vi "Define Columns.vi"(10 "enum array":refnum<vi>[](array[refnum])) -> (2 "Column Definitions":T1[](array[typedef]) {"MinWidth" min=2 step=1; "AutoSizeMode" items=["None"=1, "ColumnHeader"=2, "AllCellsExceptHeader"=4, "AllCells"=6, "DisplayedCellsExceptHeader"=8, "DisplayedCells"=10, "Fill"=16]; "FillWeight" min=1 max=100})   [LabVIEW 2015, in "Modbus Module editor node.lvclass"]
uses:
  Modbus Module editor node.lvclass
  <vilib>/NI/DCAF/Tag Editor Core/Table API/Column/Column Descriptor.ctl
  <vilib>/NI/DCAF/Tag Editor Core/Table API/Column/Column.lvclass
  <vilib>/NI/DCAF/Tag Editor Core/Table API/Column/Column Type.ctl
  <vilib>/NI/Tag Bus/tag/Data Type.ctl
  <vilib>/NI/DCAF/Tag Editor Core/Table API/Table Manager/Call Back Ref Type Def.ctl
  <vilib>/NI/DCAF/Tag Editor Core/Configuration Editor/Classes/Engine Parent/Engine Parent Editor Node.lvclass
  <vilib>/NI/DCAF/Tag Editor Core/Configuration Editor/Classes/Module editor node/module editor node.lvclass
  Callback Change Direction.vi
  CallBack Change Data Type.vi
  Callback Change Channel.vi
  <vilib>/NI/DCAF/Tag Editor Core/Table API/Mapping Column/Mapping Column.lvclass
  <vilib>/NI/DCAF/Tag Editor Core/Table API/Listbox Enum Column/List Box Enum Column.lvclass
  <vilib>/NI/DCAF/Tag Editor Core/Table API/String Column/String Column.lvclass
  <vilib>/NI/Tag Bus/tag/tag descriptor.lvclass
  <vilib>/NI/DCAF/Tag Editor Core/Table API/Table Manager/Table Manager.lvclass
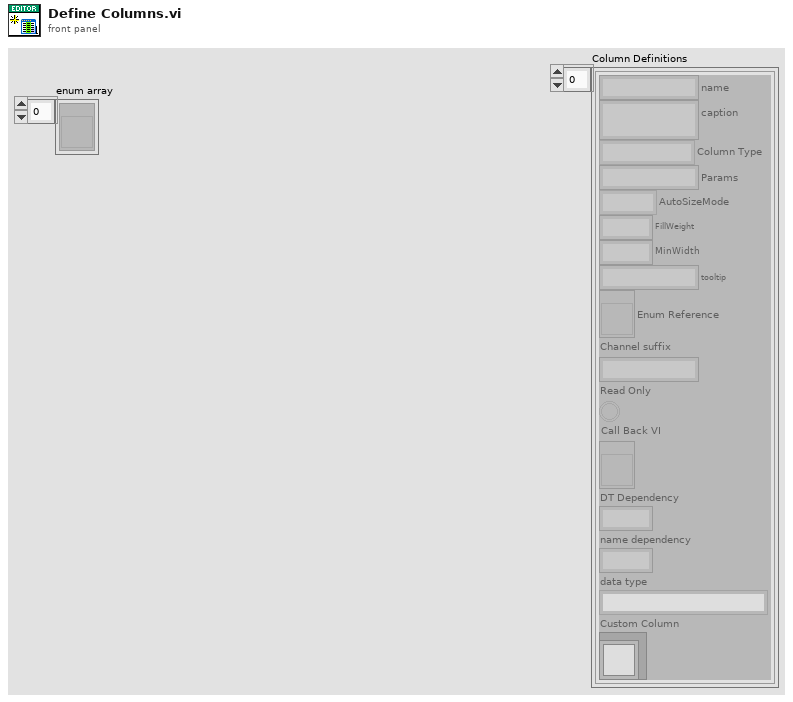
[diagram p1: front panel]
types:
  T1 = typedef "Table Manager.lvlib/Column.lvclass/Column Descriptor.ctl" = cluster{"name":string, "caption":string, "Column Type":T2, "Params":string, "AutoSizeMode":i32, "FillWeight":sgl, "MinWidth":u32, "tooltip":string, "Enum Reference":refnum<vi>, "Channel suffix":string, "Read Only":bool, "Call Back VI":T3, "DT Dependency":i32, "name dependency":i32, "data type":T4, "Custom Column":refnum<class "Column.lvclass">}
  T2 = typedef "Table Manager.lvlib/Column.lvclass/Column Type.ctl" = enum16{"String", "Mapping", "Enum", "Custom"}
  T3 = typedef "Table Manager.lvlib/Table Manager.lvclass/Call Back Ref Type Def.ctl" = refnum<vi>
  T4 = typedef "tag bus.lvlib/tag descriptor.lvclass/Data Type.ctl" = enum16{"Double", "Single", "I64", "I32", "I16", "I8", "U64", "U32", "U16", "U8", "Boolean", "String", "Array of Double", "Array of Single", "Array of I64", "Array of I32", "Array of I16", "Array of I8", "Array of U64", "Array of U32", "Array of U16", "Array of U8", "Array of Boolean", "Array of String"}
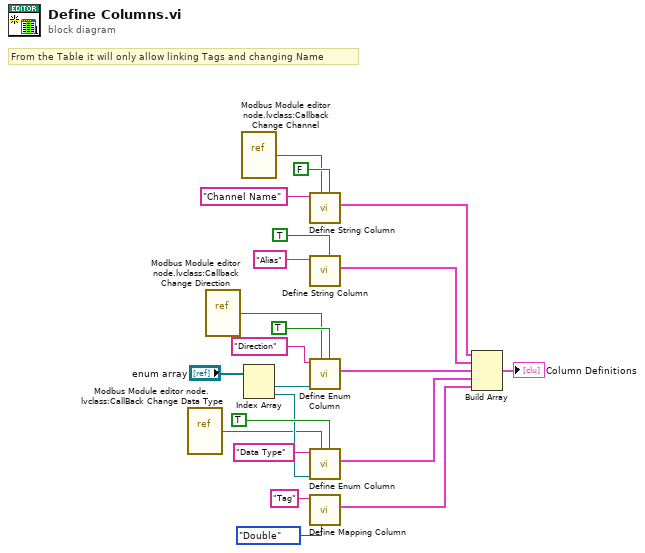
[diagram p0: block diagram]
diagram:
  # "From the Table it will only allow linking Tags and changing Name"
  n1 = vi-ref "Modbus Module editor node.lvclass:CallBack Change Data Type.vi"() -> (w8:refnum<vi>)
  n2 = vi-ref "Modbus Module editor node.lvclass:Callback Change Direction.vi"() -> (w9:refnum<vi>)
  n3 = vi-ref "Modbus Module editor node.lvclass:Callback Change Channel.vi"() -> (w7:refnum<vi>)
  n4 = Index Array(array="enum array") -> (element #1=w12:refnum<vi>, element #2=w11:refnum<vi>)  [unwired: 2 in]
  n5 = call <vilib>:"Define String Column.vi"("Read Only (F)"=FALSE ("Read Only"), "Call Back VI"=w7, "Name"="Channel Name") -> ("Column Descriptor out"=w6:T1)  [unwired: 8 in]
  n6 = call <vilib>:"Define String Column.vi"("Read Only (F)"=TRUE ("Read Only"), "Name"="Alias") -> ("Column Descriptor out"=w5:T1)  [unwired: 9 in]
  n7 = call <vilib>:"Define Enum Column.vi"("Read Only (F)"=TRUE ("Read Only"), "Call Back VI"=w9, "Enum Reference"=w12, "Name"="Direction") -> ("Column Descriptor out"=w4:T1)  [unwired: 7 in]
  n8 = call <vilib>:"Define Enum Column.vi"("Read Only (F)"=TRUE ("Read Only"), "Call Back VI"=w8, "Enum Reference"=w11, "Name"="Data Type") -> ("Column Descriptor out"=w3:T1)  [unwired: 7 in]
  n9 = call <vilib>:"Define Mapping Column.vi"("data type"=Data_Type."Double", "name"="Tag") -> ("Column Descriptor out"=w2:T1)  [unwired: 9 in]
  n10 = Build Array(w6, w5, w4, w3, w2) -> (→"Column Definitions":T1[])
